vi "VIH Utility - STR - Filter 1D Array of Strings.vi"(6 "Action (keep instances)":enum16{"keep instances", "remove instances"}(ring), 8 "error in":errorcluster, 9 "case-sencitive (T)":bool=TRUE, 10 "instances":string[](array[string]), 11 "Array in":string[](array[string])) -> (0 "error out":errorcluster, 3 "Array out":string[](array[string]))   [LabVIEW 2014]
doc: "::: VI Helpeks :::\nCopyright (c) 2000-2026 Konstantin Shifershteyn. All rights reserved."
panel:
  # "VI Helpeks\nCopyright (c) 2012-2026 Konstantin Shifershteyn"
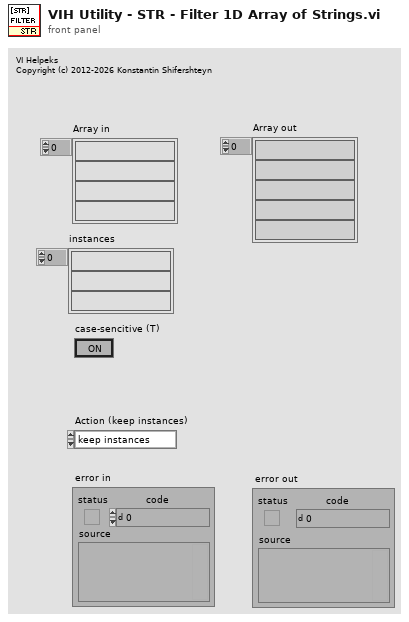
[diagram p1: front panel]
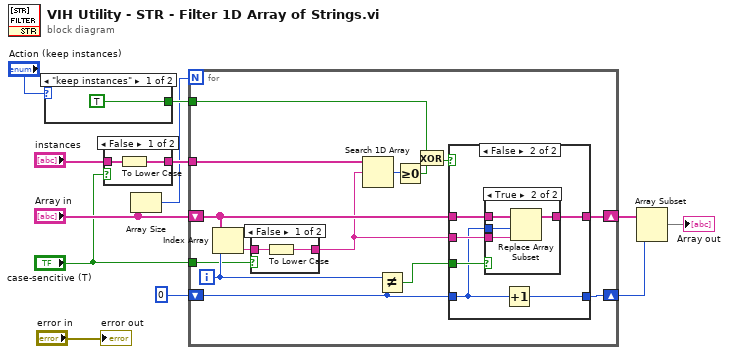
[diagram p0: block diagram]
diagram:
  n1 = case shown="\"keep instances\"" "Action (keep instances)" {
    tunnel: [TRUE _] -> w8
    frame "keep instances" {
    }
    frame "remove instances" {
    }
  }
  n2 = case shown="False" "case-sencitive (T)" {
    tunnel: "instances" -> [w15 w16]
    tunnel: [w14 w16] -> w6
    frame False {
      n3 = To Lower Case(string=w15) -> (all lower case string=w14:string[])
    }
    frame True {
    }
  }
  n4 = Array Size(array="Array in") -> (size(s)=w4:i32)
  n5 = for {
    N: w4 -> [_]
    tunnel: w6 -> [w30]
    shift-right: [w28] -> w12
    shift-left: "Array in" -> [w20]
    shift-right: [w29] -> w1
    shift-left: 0 -> [w26]
    tunnel: w8 -> [w24]
    tunnel: "case-sencitive (T)" -> [w17]
    i -> [w21]
    n6 = Index Array(array=w20, index=w21) -> (element=w19:string)
    n7 = case shown="False" w17 {
      tunnel: w19 -> [w32 w33]
      tunnel: [w31 w33] -> w18
      frame False {
        n8 = To Lower Case(string=w32) -> (all lower case string=w31:string)
      }
      frame True {
      }
    }
    n9 = Search 1D Array(1D array=w30, element=w18) -> (index of element=w23:i32)  [unwired: 1 out]
    n10 = Not Equal?(x=w21, y=w26) -> (x != y?=w27:bool)
    n11 = Greater Or Equal To 0?(x=w23) -> (x >= 0?=w25:bool)
    n12 = Exclusive Or(1:w25, 2:w24) -> (0:w22:bool)
    n13 = case shown="False" w22 {
      tunnel: w20 -> [w35 w41]
      tunnel: w18 -> [_ w40]
      tunnel: w26 -> [w34 w37]
      tunnel: [w34 w36] -> w29
      tunnel: [w35 w39] -> w28
      tunnel: w27 -> [_ w38]
      frame True {
      }
      frame False {
        n14 = case shown="True" w38 {
          tunnel: w41 -> [w42 w46]
          tunnel: w40 -> [_ w45]
          tunnel: [w42 w44] -> w39
          tunnel: w37 -> [_ w43]
          frame False {
          }
          frame True {
            n15 = Replace Array Subset(array=w46, new element=w45, index=w43) -> (w44:string[])
          }
        }
        n16 = Increment(x=w37) -> (x+1=w36:i32)
      }
    }
  }
  n17 = Array Subset(array=w12, length=w1) -> (→"Array out":string[])  [unwired: 1 in]
  "error out" <- "error in"
